vi "Update.vi"(8 "error in (no error)":errorcluster, 11 "GroupLoggingControl in":refnum<class "GroupLoggingControl.lvclass">) -> (0 "error out":errorcluster, 3 "GroupLoggingControl out":refnum<class "GroupLoggingControl.lvclass">)   [LabVIEW 2020, in "VolatusGUIElements.lvlib" / "GroupLoggingControl.lvclass"]
uses:
  GroupLoggingControl.lvclass
  C:/dev/lv20CE/relink/lv-volatus/VolatusGUI/GUI Element/GUI Element.lvclass
  VolatusGUI/GUI Element/GUI Element.lvclass/GUI Element.ctl
  GroupLoggingControl.lvclass/GroupLoggingControl.ctl
  <vilib>/Utility/miscctls.llb/LVMapReplaceAction.ctl
  lv-vecto/Vecto/Channel DBL/Channel DBL.lvclass/Channel DBL.ctl
  lv-vecto/Vecto/Group DBL/Value by Index.vi
  lv-vecto/Vecto/Channel DBL/Channel DBL.lvclass
  Volatus/VolatusAPI/VolatusAPI.lvclass
  <vilib>/httpClient/LabVIEWHTTPClient.lvlib
  VolatusGUI/GUI Element/GUI Element.lvclass
panel:
  out "error out 2":errorcluster
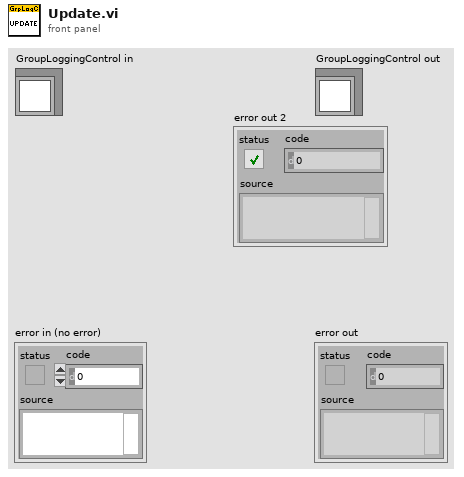
[diagram p1: front panel]
types:
  T1 = cluster{"Series":string, "Timestamp":string, "Targets":cluster{"Node":string, "Node Color":u32, "Groups":cluster{"Group":string, "Group Color":u32, "Button":bool}[]}[], "Groups":cluster{"Group":string, "Group Color":u32, "Button":bool}[]}
  T2 = cluster{"Group":string, "Group Color":u32, "Button":bool}[]
  T3 = typedef "VolatusGUIElements.lvlib/GroupLoggingControl.lvclass/Status.ctl" = cluster{"Groups":T4[], "Targets":T7[]}
  T4 = typedef "VolatusGUIElements.lvlib/GroupLoggingControl.lvclass/Log Group.ctl" = cluster{"Status":T5, "Command Info":T6, "Logging":bool, "State":string}
  T5 = typedef "VolatusGUIElements.lvlib/GroupLoggingControl.lvclass/Log Group Status.ctl" = cluster{"Group":string, "Group Color":u32, "Button":bool}
  T6 = typedef "VolatusGUIElements.lvlib/GroupLoggingControl.lvclass/Command Info.ctl" = cluster{"Commanding":bool, "Cmd Time":dbl, "Group ID":string}
  T7 = typedef "VolatusGUIElements.lvlib/GroupLoggingControl.lvclass/Target Info.ctl" = cluster{"Node":string, "Node Color":u32, "Groups":T4[]}
  T8 = typedef "LVMapReplaceAction.ctl" = enum32{"Modify Entry only if found", "Add or Modify Entry", "Delete Entry"}
  T9 = cluster{"State":string, "Log":string, "Groups":cluster{"Group":string, "State":string}[]}
  T10 = cluster{"Group":string, "Group Color":u32, "Button":bool}
  T11 = cluster{"Node":string, u32, cluster{"Group":string, "Group Color":u32, "Button":bool}[]}
  T12 = cluster{string, string, cluster{"Node":string, u32, cluster{"Group":string, "Group Color":u32, "Button":bool}[]}[], "Groups":cluster{"Group":string, "Group Color":u32, "Button":bool}[]}
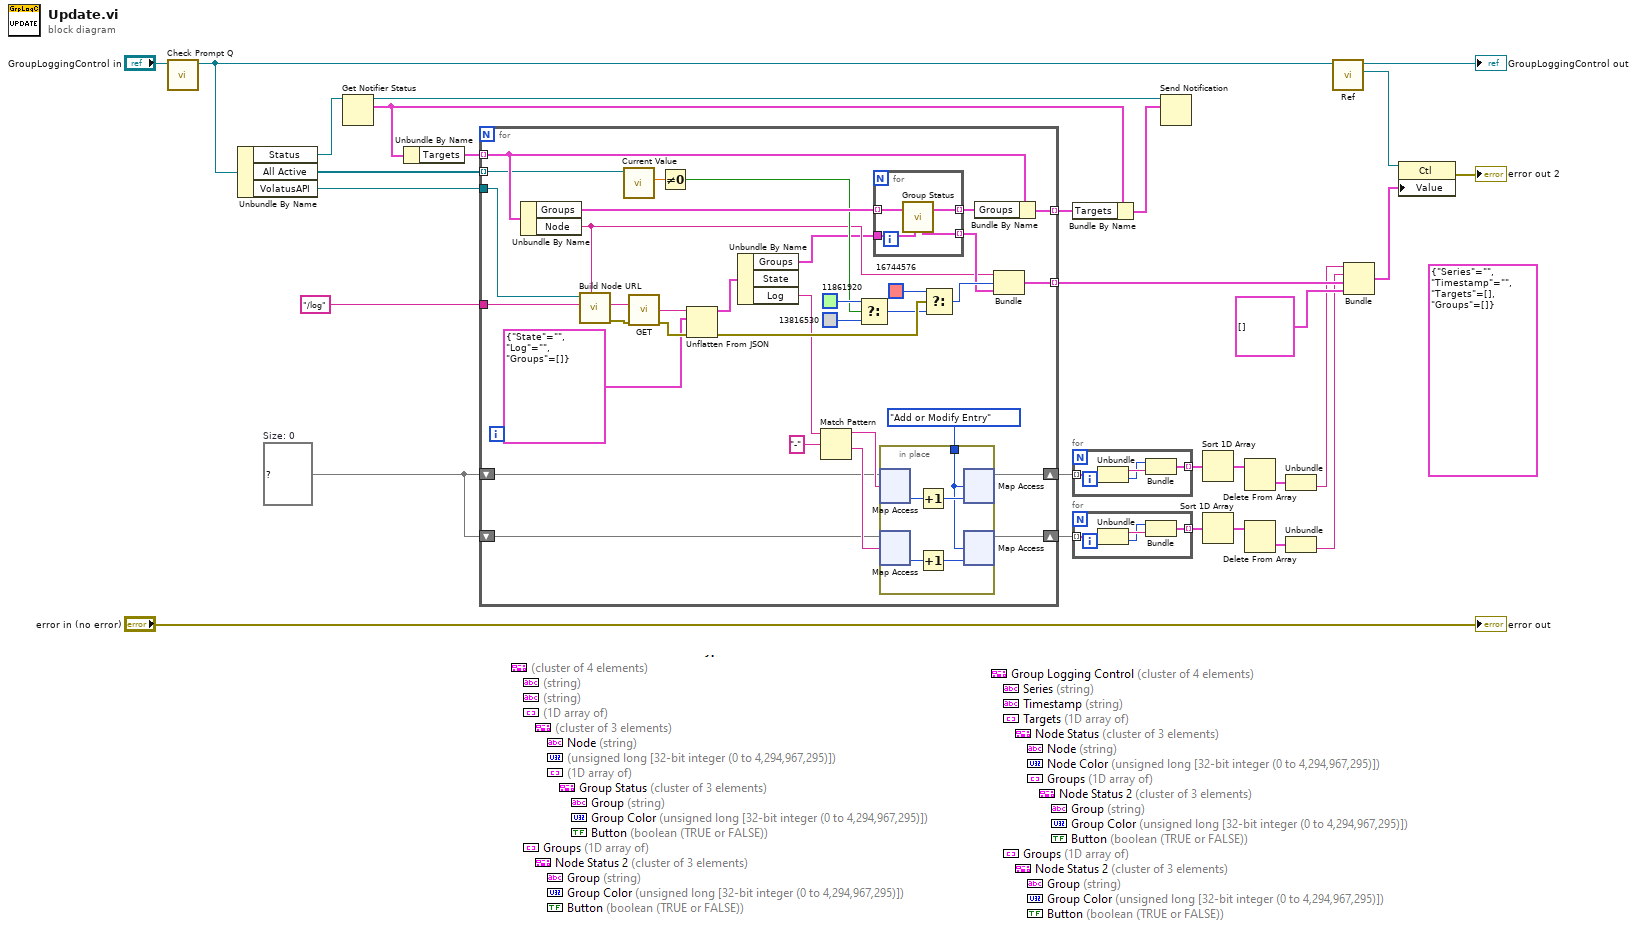
[diagram p0: block diagram]
diagram:
  (unwired) T1 {"Series"="", "Timestamp"="", "Targets"=[], "Groups"=[]} ("Group Logging Control")
  w24 = map{string, i32} {}  # Size: 0
  n1 = call "Check Prompt Q.vi"("LoggingControl in"="GroupLoggingControl in") -> ("LoggingControl out"=w1:refnum<class "GroupLoggingControl.lvclass">)  [unwired: 9 in, 1 out]
  n2 = Unbundle By Name(w1) -> ("Status"=w6:refnum<notifier>, "All Active"=w25:refnum<class "Channel DBL.lvclass">[], "VolatusAPI"=w23:refnum<class "VolatusAPI.lvclass">)
  n3 = Get Notifier Status(notifier=w6) -> (notifier out=w3:refnum<notifier>, current notification=w4:T3)  [unwired: 1 in, 3 out]
  n4 = Unbundle By Name(w4) -> ("Targets"=w5:T7[])
  n5 = for {
    tunnel: w5 -> [w54] mode=indexing
    tunnel: [w57] -> w28 mode=indexing
    tunnel: [w52] -> w21 mode=indexing
    tunnel: w25 -> [w50] mode=indexing
    shift-right: [w33] -> w14
    shift-left: w24 -> [w32]
    shift-right: [w34] -> w13
    shift-left: w24 -> [w31]
    tunnel: w23 -> [w43]
    tunnel: "/log" -> [w41]
    n6 = Unbundle By Name(w54) -> ("Groups"=w56:T4[], "Node"=w42:string)
    n7 = call "Build Node URL.vi"("Node Name"=w42, "Path"=w41, "VolatusAPI in"=w43) -> ("error out"=w48:errorcluster, "Request URL"=w46:string)  [unwired: 6 in, 1 out]
    n8 = call "Current Value.vi"("Channel in"=w50) -> ("Scaled"=w51:dbl)  [unwired: 6 in, 4 out]
    n9 = call <vilib>:"GET.vi"("url"=w46, "error in (no error)"=w48) -> ("body"=w47:string, "error out"=w45:errorcluster)  [unwired: 10 in, 2 out]
    n10 = Not Equal To 0?(x=w51) -> (x != 0?=w49:bool)
    n11 = Unflatten From JSON(JSON string=w47, type and defaults=T9 {"State"="", "Log"="", "Groups"=[]} ("output cluster"), error in (no error)=w45) -> (value=w36:T9, error out=w63:errorcluster)  [unwired: 4 in]
    n12 = Unbundle By Name(w36) -> ("Groups"=w30:cluster{"Group":string, "State":string}[], "Log"=w35:string)  [unwired: 1 out]
    n13 = Match Pattern(string=w35, regular expression="-") -> (before substring=w38:string, after substring=w37:string)  [unwired: 1 in, 2 out]
    n14 = Select(t=u32 11861920, s=w49, f=u32 13816530) -> (s? t:f=w60:u32)
    n15 = for {
      tunnel: w56 -> [w72] mode=indexing
      tunnel: [w71] -> w55 mode=indexing
      tunnel: [w70] -> w53 mode=indexing
      tunnel: w30 -> [w69]
      n16 = call "Group Status.vi"("Log Group"=w72, "Groups"=w69) -> ("Group Status"=w71:T10, "Group"=w70:T4)  [unwired: 4 in]
    }
    n17 = in-place {
      in-place-border: LVMapReplaceAction."Add or Modify Entry" ("action") -> [w64]
      n18 = in-place-map #1(w32, w38) -> (w68:i32)  [unwired: 1 in, 1 out]
      n19 = in-place-map #2(w31, w37) -> (w67:i32)  [unwired: 1 in, 1 out]
      n20 = Increment(x=w68) -> (x+1=w65:i32)
      n21 = Increment(x=w67) -> (x+1=w66:i32)
      n22 = in-place-map #1(w65, w64) -> (w33:map{string, i32})  [unwired: 2 out]
      n23 = in-place-map #2(w66, w64) -> (w34:map{string, i32})  [unwired: 2 out]
    }
    n24 = Select(t=u32 16744576, s=w63, f=w60) -> (s? t:f=w58:u32)
    n25 = Bundle By Name(cluster=w54, "Groups"=w53) -> (w52:T7)
    n26 = Bundle("Node"=w42, w58, w55) -> (w57:T11)  [unwired: 1 in]
  }
  n27 = Bundle By Name(cluster=w4, "Targets"=w21) -> (w2:T3)
  n28 = for {
    tunnel: w14 -> [w76] mode=indexing
    tunnel: [w73] -> w20 mode=indexing
    n29 = Unbundle(w76) -> (w75:string, w74:i32)
    n30 = Bundle(w74, w75) -> (w73:cluster{i32, string})  [unwired: 1 in]
  }
  n31 = for {
    tunnel: w13 -> [w80] mode=indexing
    tunnel: [w77] -> w15 mode=indexing
    n32 = Unbundle(w80) -> (w79:string, w78:i32)
    n33 = Bundle(w78, w79) -> (w77:cluster{i32, string})  [unwired: 1 in]
  }
  n34 = Send Notification(notification=w2, notifier=w3) -> ()  [unwired: 1 in, 2 out]
  n35 = Sort 1D Array(array=w20) -> (sorted array=w19:cluster{i32, string}[])
  n36 = Sort 1D Array(array=w15) -> (sorted array=w16:cluster{i32, string}[])
  n37 = Delete From Array(array=w19) -> (deleted portion=w18:cluster{i32, string})  [unwired: 2 in, 1 out]
  n38 = Delete From Array(array=w16) -> (deleted portion=w17:cluster{i32, string})  [unwired: 2 in, 1 out]
  n39 = Unbundle(w18) -> (w12:string)  [unwired: 1 out]
  n40 = Unbundle(w17) -> (w11:string)  [unwired: 1 out]
  n41 = call "Ref.vi"("GUI Element in"=w1) -> ("Ref"=w9:refnum<vi>, "GUI Element out"=→"GroupLoggingControl out":refnum<class "GroupLoggingControl.lvclass">)  [unwired: 9 in]
  n42 = Bundle(w12, w11, w28, "Groups"=T2 []) -> (w8:T12)  [unwired: 1 in]
  n43 = property class="Ctl"(reference=w9, "Value"=w8) -> (error out=→"error out 2":errorcluster)  [unwired: 1 in, 1 out]
  "error out" <- "error in (no error)"
